vi "set Modulation Index Table Type.vi"(8 "error in (no error)":errorcluster, 9 "Direction":T2, 10 "Modulation Table":T1, 11 "NR in":refnum<class "NR.lvclass">) -> (0 "error out":errorcluster, 3 "NR out":refnum<class "NR.lvclass">)   [LabVIEW 2023, in "ANRITSU Call Box.lvlib" / "NR.lvclass"]
uses:
  NR.lvclass
  NR.lvclass/NR.ctl
  Type Definition/Uplink Downlink Enum.ctl
  ANRITSU Call Box.lvlib
  Type Definition/Modulation Table Selector.ctl
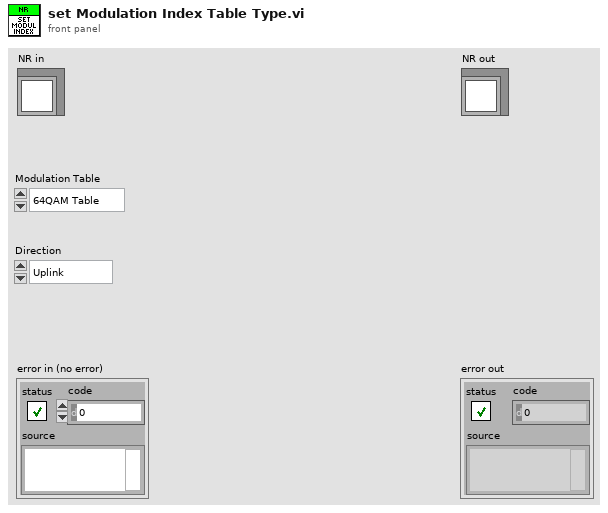
[diagram p1: front panel]
types:
  T1 = typedef "ANRITSU Call Box.lvlib/Modulation Table Selector.ctl" = enum16{"64QAM Table", "256QAM Table"}
  T2 = typedef "ANRITSU Call Box.lvlib/Uplink Downlink Enum.ctl" = enum16{"Uplink", "Downlink"}
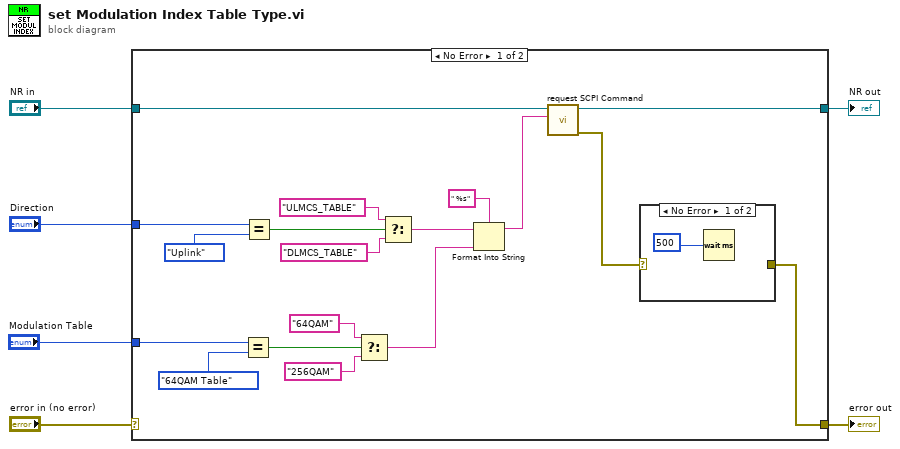
[diagram p0: block diagram]
diagram:
  n1 = case shown="No Error" "error in (no error)" {
    selector: "error in (no error)" -> [_ w28]
    tunnel: [w8 w28] -> w5
    tunnel: [w7 w27] -> w3
    tunnel: "NR in" -> [w11 w27]
    tunnel: "Direction" -> [w24 _]
    tunnel: "Modulation Table" -> [w19 _]
    frame No Error {
      n2 = Equal?(x=w19, y=Modulation_Table_Selector."64QAM Table") -> (x = y?=w15:bool)
      n3 = Equal?(x=w24, y=Uplink_Downlink_Enum."Uplink") -> (x = y?=w20:bool)
      n4 = Select(t="64QAM", s=w15, f="256QAM") -> (s? t:f=w12:string)
      n5 = Select(t="ULMCS_TABLE", s=w20, f="DLMCS_TABLE") -> (s? t:f=w13:string)
      n6 = Format Into String(format string=" %s", initial string=w13, w12) -> (resulting string=w10:string)  [unwired: 1 in, 1 out]
      n7 = call "request SCPI Command.vi"("SCPI Command"=w10, "NR in"=w11) -> ("error out"=w9:errorcluster, "NR out"=w7:refnum<class "NR.lvclass">)  [unwired: 8 in]
      n8 = case shown="No Error" w9 {
        selector: w9 -> [_ w26]
        tunnel: [_ w26] -> w8
        frame No Error {
          n9 = Wait (ms)(milliseconds to wait=u32 500) -> ()  [unwired: 1 out]
        }
        frame Error {
        }
      }
    }
    frame Error {
    }
  }
  "error out" <- w5
  "NR out" <- w3
